vi "testRun.vi"() -> ()   [LabVIEW 2025, in "H1VelocityTest.lvclass"]
uses:
  H1VelocityTest.lvclass
  H1VelocityTest.lvclass/H1VelocityTest.ctl
  H1 Velocity.lvclass
  <vilib>/measure/NI_MABase.lvlib
panel:
  in  "loop":u32=50
  in  "Test":T1(ring)=enum."Centering"
  # "Not exceed 50 ms"
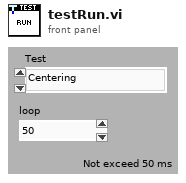
[diagram p1: front panel]
types:
  T1 = enum16{"Loaded Velocity", "Piston Velocity", "Centering"}
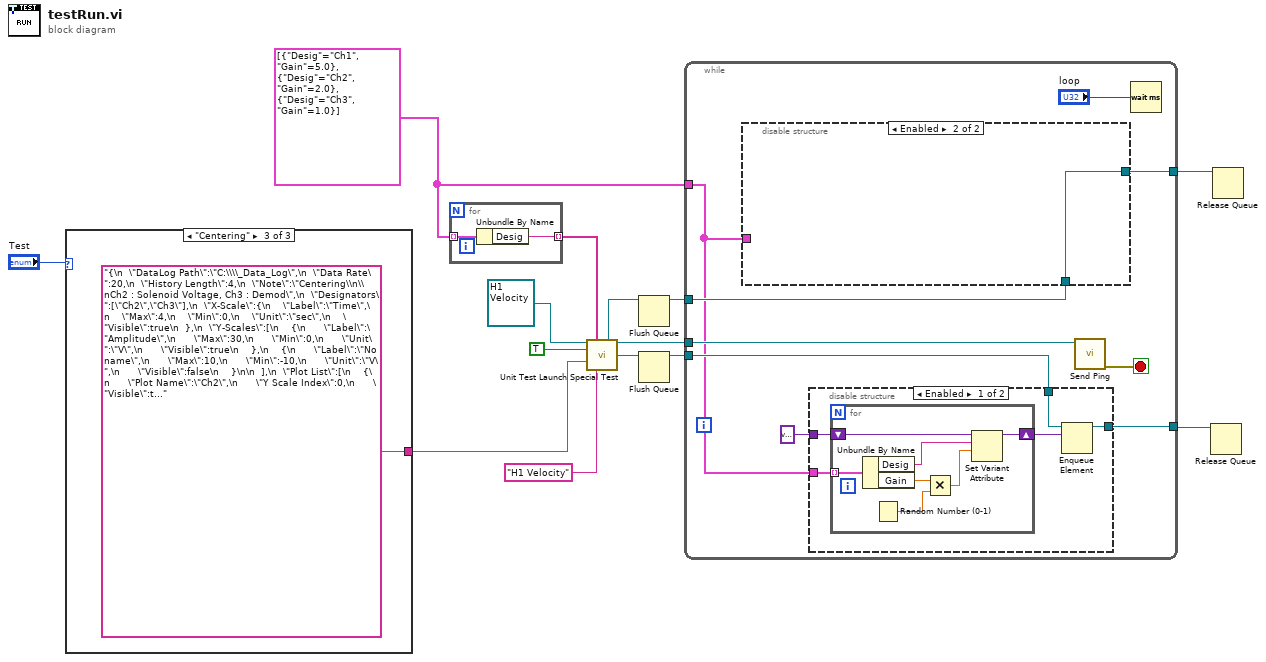
[diagram p0: block diagram]
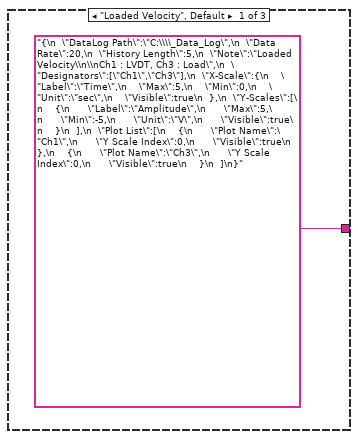
[diagram p2: hidden frame]
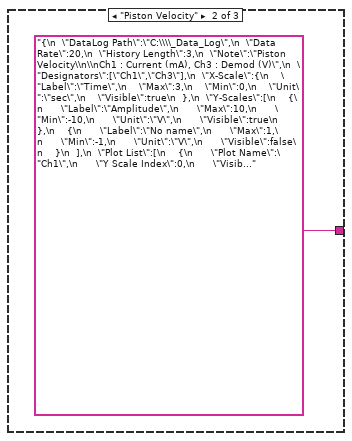
[diagram p3: hidden frame]
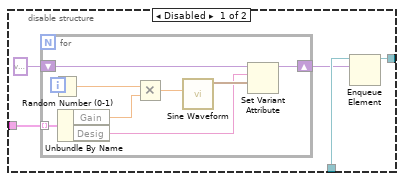
[diagram p4: hidden frame]
diagram:
  w3 = cluster{"Desig":string, "Gain":dbl}[] [{"Desig"="Ch1", "Gain"=5.0}, {"Desig"="Ch2", "Gain"=2.0}, {"Desig"="Ch3", "Gain"=1.0}] ("Sim Param")
  n1 = case shown="\"Centering\"" "Test" {
    tunnel: ["{\n  \"DataLog Path\":\"C:\\\\_Data_Log\",\n  \"Data Rate\":20,\n  \"History Length\":5,\n  \"Note\":\"Loaded Velocity\\n\\nCh1 : LVDT, Ch3 : Load\",\n  \"Designators\":[\"Ch1\",\"Ch3\"],\n  \"X-Scale\":{\n    \"Label\":\"Time\",\n    \"Max\":5,\n    \"Min\":0,\n    \"Unit\":\"sec\",\n    \"Visible\":true\n  },\n  \"Y-Scales\":[\n    {\n      \"Label\":\"Amplitude\",\n      \"Max\":5,\n      \"Min\":-5,\n      \"Unit\":\"V\",\n      \"Visible\":true\n    }\n  ],\n  \"Plot List\":[\n    {\n      \"Plot Name\":\"Ch1\",\n      \"Y Scale Index\":0,\n      \"Visible\":true\n    },\n    {\n      \"Plot Name\":\"Ch3\",\n      \"Y Scale Index\":0,\n      \"Visible\":true\n    }\n  ]\n}" ("Settings_JSON_") "{\n  \"DataLog Path\":\"C:\\\\_Data_Log\",\n  \"Data Rate\":20,\n  \"History Length\":3,\n  \"Note\":\"Piston Velocity\\n\\nCh1 : Current (mA), Ch3 : Demod (V)\",\n  \"Designators\":[\"Ch1\",\"Ch3\"],\n  \"X-Scale\":{\n    \"Label\":\"Time\",\n    \"Max\":3,\n    \"Min\":0,\n    \"Unit\":\"sec\",\n    \"Visible\":true\n  },\n  \"Y-Scales\":[\n    {\n      \"Label\":\"Amplitude\",\n      \"Max\":10,\n      \"Min\":-10,\n      \"Unit\":\"V\",\n      \"Visible\":true\n    },\n    {\n      \"Label\":\"No name\",\n      \"Max\":1,\n      \"Min\":-1,\n      \"Unit\":\"V\",\n      \"Visible\":false\n    }\n  ],\n  \"Plot List\":[\n    {\n      \"Plot Name\":\"Ch1\",\n      \"Y Scale Index\":0,\n      \"Visible\":true\n    },\n    {\n      \"Plot Name\":\"Ch3\",\n      \"Y Scale Index\":0,\n      \"Visible\":true\n    }\n  ]\n}" ("Settings_JSON_") "{\n  \"DataLog Path\":\"C:\\\\_Data_Log\",\n  \"Data Rate\":20,\n  \"History Length\":4,\n  \"Note\":\"Centering\\n\\nCh2 : Solenoid Voltage, Ch3 : Demod\",\n  \"Designators\":[\"Ch2\",\"Ch3\"],\n  \"X-Scale\":{\n    \"Label\":\"Time\",\n    \"Max\":4,\n    \"Min\":0,\n    \"Unit\":\"sec\",\n    \"Visible\":true\n  },\n  \"Y-Scales\":[\n    {\n      \"Label\":\"Amplitude\",\n      \"Max\":30,\n      \"Min\":0,\n      \"Unit\":\"V\",\n      \"Visible\":true\n    },\n    {\n      \"Label\":\"No name\",\n      \"Max\":10,\n      \"Min\":-10,\n      \"Unit\":\"V\",\n      \"Visible\":false\n    }\n\n  ],\n  \"Plot List\":[\n    {\n      \"Plot Name\":\"Ch2\",\n      \"Y Scale Index\":0,\n      \"Visible\":true\n    },\n    {\n      \"Plot Name\":\"Ch3\",\n      \"Y Scale Index\":1,\n      \"Visible\":true\n    }\n  ]\n}" ("Settings_JSON_")] -> w10
    frame "Loaded Velocity", Default {
    }
    frame "Piston Velocity" {
    }
    frame "Centering" {
    }
  }
  n2 = for {
    tunnel: w3 -> [w19] mode=indexing
    tunnel: [w18] -> w12 mode=indexing
    n3 = Unbundle By Name(w19) -> ("Desig"=w18:string)
  }
  n4 = call "Unit Test Launch Special Test.vi"("Special Test Class"=refnum<class "H1 Velocity.lvclass"> refnum ("Sensitivity.lvlib:Sensitivity.lvclass"), "Subscription Alias"=w12, "Auto Launched"=TRUE, "<JSON>"=w10, "Debug Alias"="H1 Velocity") -> ("Data Queue out"=w2:refnum<queue>, "ST Enqueuer out"=w4:refnum<class "Message Enqueuer.lvclass">, "Fast Map Queue out"=w5:refnum<queue>)  [unwired: 2 in, 6 out]
  n5 = Flush Queue(queue=w2) -> (queue out=w8:refnum<queue>)  [unwired: 1 in, 2 out]
  n6 = Flush Queue(queue=w5) -> (queue out=w9:refnum<queue>)  [unwired: 1 in, 2 out]
  n7 = while {
    tunnel: w4 -> [w28]
    tunnel: w9 -> [w25]
    tunnel: [w23] -> w6
    tunnel: w3 -> [w22]
    tunnel: w8 -> [w27]
    tunnel: [w24] -> w7
    stop <- w21 stop-if-true
    n8 = disable-structure shown="Enabled" {
      disable-tunnel: w27 -> [w32 w42]
      disable-tunnel: [w31 w42] -> w23
      disable-tunnel: w22 -> [w30 _]
      frame Disabled {
        n9 = for {
          shift-right: [w40] -> w29
          shift-left: variant ("variant") -> [w41]
          tunnel: w30 -> [w38] mode=indexing
          n10 = Random Number (0-1)() -> (number: 0 to 1=w34:dbl)
          n11 = Unbundle By Name(w38) -> ("Gain"=w36:dbl, "Desig"=w37:string)
          n12 = Multiply(x=w34, y=w36) -> (x*y=w35:dbl)
          n13 = call <vilib>:"Sine Waveform.vi"("amplitude"=w35) -> ("signal out"=w39:waveform(dbl))  [unwired: 9 in, 1 out]
          n14 = Set Variant Attribute(Variant=w41, name=w37, value=w39) -> (Variant out=w40:variant)  [unwired: 1 in, 2 out]
        }
        n15 = Enqueue Element(queue=w32, element=w29) -> (queue out=w31:refnum<queue>)  [unwired: 2 in, 2 out]
      }
      frame Enabled {
      }
    }
    n16 = disable-structure shown="Enabled" {
      disable-tunnel: variant ("variant") -> [w47 _]
      disable-tunnel: w25 -> [w46 w55]
      disable-tunnel: [w45 w55] -> w24
      disable-tunnel: w22 -> [w44 _]
      frame Enabled {
        n17 = for {
          shift-right: [w53] -> w43
          shift-left: w47 -> [w54]
          tunnel: w44 -> [w52] mode=indexing
          n18 = Unbundle By Name(w52) -> ("Desig"=w51:string, "Gain"=w50:dbl)
          n19 = Random Number (0-1)() -> (number: 0 to 1=w49:dbl)
          n20 = Multiply(x=w50, y=w49) -> (x*y=w48:dbl)
          n21 = Set Variant Attribute(Variant=w54, name=w51, value=w48) -> (Variant out=w53:variant)  [unwired: 1 in, 2 out]
        }
        n22 = Enqueue Element(queue=w46, element=w43) -> (queue out=w45:refnum<queue>)  [unwired: 2 in, 2 out]
      }
      frame Disabled {
      }
    }
    n23 = call "Send Ping.vi"("Message Enqueuer"=w28) -> ("error out"=w21:errorcluster)  [unwired: 6 in, 4 out]
    n24 = Wait (ms)(milliseconds to wait="loop") -> ()  [unwired: 1 out]
  }
  n25 = Release Queue(queue=w7) -> ()  [unwired: 2 in, 3 out]
  n26 = Release Queue(queue=w6) -> ()  [unwired: 2 in, 3 out]
